vi "FULL_ADDER.vi"() -> ()   [LabVIEW 2018]
panel:
  in  "C":bool
  out "COUT 4":bool
  out "SUM 3":bool
  in  "B":bool
  in  "A":bool
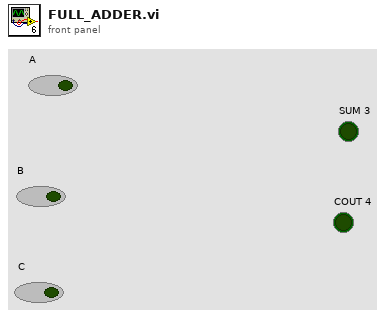
[diagram p1: front panel]
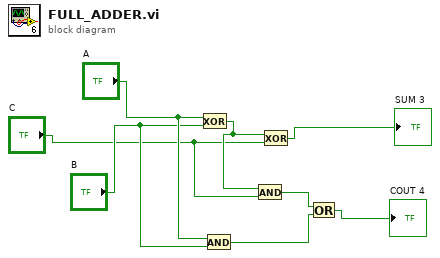
[diagram p0: block diagram]
diagram:
  n1 = Exclusive Or(1:"B", 2:"A") -> (0:w6:bool)
  n2 = And(x="A", y="B") -> (x .and. y?=w3:bool)
  n3 = And(x=w6, y="C") -> (x .and. y?=w4:bool)
  n4 = Exclusive Or(1:"C", 2:w6) -> (0:→"SUM 3":bool)
  n5 = Or(x=w4, y=w3) -> (x .or. y?=→"COUT 4":bool)
